vi "2636 Pulse Generator.vi"() -> ()   [LabVIEW 2023]
uses:
  <instrlib>/Keithley 2600 Series/Public/Channel.ctl
  <instrlib>/Keithley 2600 Series/Keithley 2600 Series.lvlib
  <userlib>/_OpenG.lib/time/time.llb/openg_time.lvlib
panel:
  in  "Pulse Number":u32=10
  out "Gate Pulse":cluster{"X":dbl[], "Y":dbl[]}[](graph)
  in  "error in (no error)":errorcluster
  in  "Auto Enable Output":bool=TRUE
  in  "Reset":bool=TRUE
  in  "Error Query":bool
  out "error out":errorcluster
  out "Complete?":bool
  in  "Stop":bool
  in  "Pulse Duration (s)":dbl=0.01
  in  "Post-Pulse Duration (s)":dbl=0.05
  in  "Pre-Pulse Duration (s)":dbl=0.05
  in  "Pulse Level (V)":dbl=15.0
  in  "Pulse Channel":T1
  in  "2636 Address":refnum<visa-resource-name>="GPIB0::26::INSTR"
  # "Pulse Generator"
  # "by JHC (20250611)"
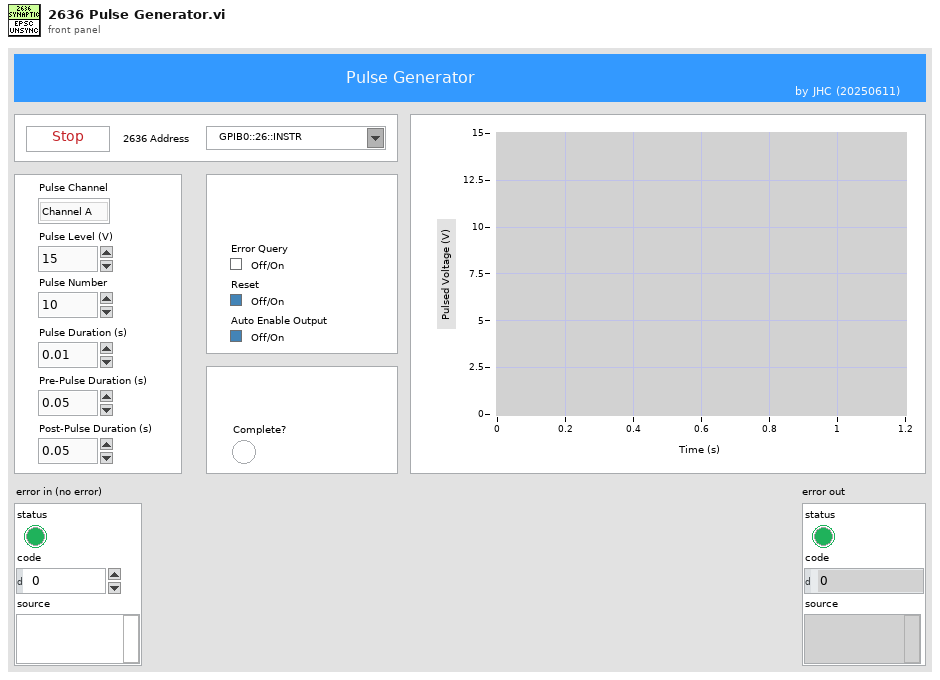
[diagram p1: front panel]
types:
  T1 = typedef "Keithley 2600 Series.lvlib/Channel.ctl" = enum32{"Channel A", "Channel B"}
  T2 = enum16{"None/Disconnect", "Digital I/O Trigger", "TSP-Link Trigger", "LAN Trigger", "Blender", "Timer Expired", "Front Panel Trigger", "Software Trigger", "SMU Sweeping", "SMU Armed", "SMU Source Complete", "SMU Measure Complete", "SMU Pulse Complete", "SMU Sweep Complete", "SMU Idle"}
  T3 = enum16{"Current", "Voltage", "IV", "Resistance", "Power"}
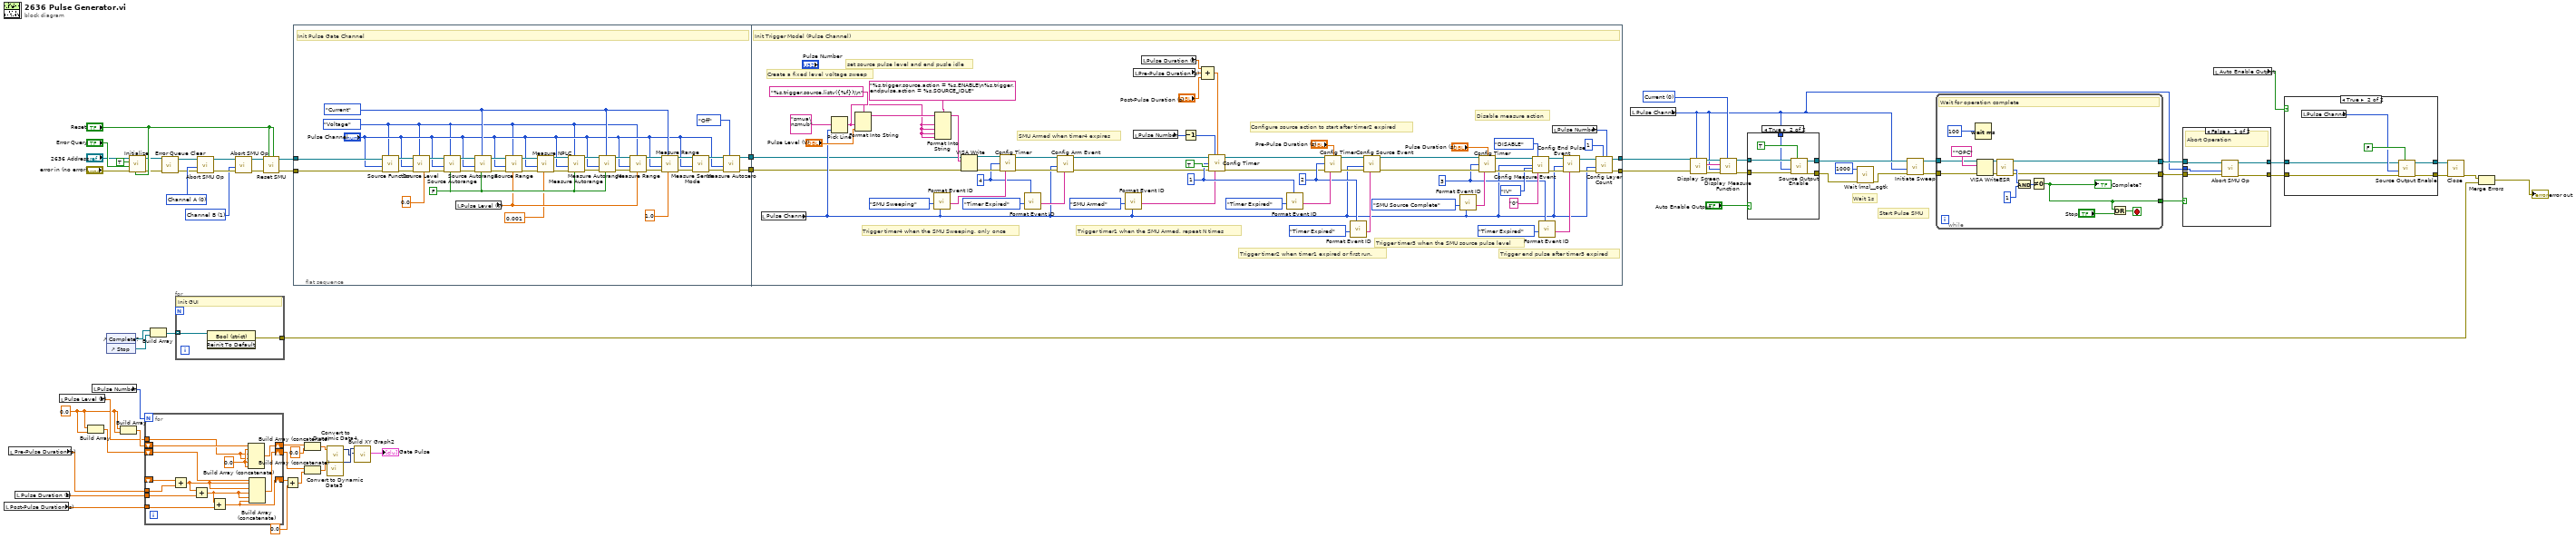
[diagram p0: block diagram]
diagram:
  w6 = 0.0 ("element")
  w42 = u16 1 items=["Channel A", "Channel B"] ("Channel (Channel A)")
  w43 = u16 0 items=["Channel A", "Channel B"] ("Channel (Channel A)")
  w52 = u16 0 items=["Current", "Voltage", "Resistance", "Power"] ("Function (Current)")
  # "Wait 1s"
  # "Start Pulse SMU"
  n1 = local read "Post-Pulse Duration (s)"() -> (w19:dbl)
  n2 = local read "Pre-Pulse Duration (s)"() -> (w22:dbl)
  n3 = local read "Pulse Duration (s)"() -> (w20:dbl)
  n4 = local read "Pulse Level (V)"() -> (w21:dbl)
  n5 = Build Array(w6, w6) -> (w24:dbl[])
  n6 = local read "Pulse Number"() -> (w25:u32)
  n7 = control-ref of="Complete?"() -> (w50:refnum<vi>)
  n8 = control-ref of="Stop"() -> (w48:refnum<vi>)
  n9 = Build Array(w6, w6) -> (w23:dbl[])
  n10 = call <instrlib>:"Initialize.vi"("Reset (True)"="Reset", "error in (no error)"="error in (no error)", "Error Query (False)"="Error Query", "ID Query (True)"=TRUE, "VISA resource name"="2636 Address") -> ("error out"=w27:errorcluster, "VISA resource name out"=w30:refnum<visa-resource-name>)  [unwired: 5 in]
  n11 = for {
    N: w25 -> [_]
    shift-right: [w77] -> w18
    shift-left: w23 -> [w78]
    shift-right: [w79] -> w17
    shift-left: w24 -> [w80]
    tunnel: w22 -> [w74]
    tunnel: w21 -> [w69]
    tunnel: w20 -> [w76]
    shift-right: [w71] -> w10
    shift-left: _ -> [w81]
    tunnel: w19 -> [w75]
    w73 = 0.0 ("element")
    n12 = Add(x=w81, y=w74) -> (x+y=w72:dbl)
    n13 = Add(x=w72, y=w76) -> (x+y=w70:dbl)
    n14 = Add(x=w70, y=w75) -> (x+y=w71:dbl)
    n15 = Build Array (concatenate)(w78, w73, w69, w69, w73, w73) -> (w77:dbl[])
    n16 = Build Array (concatenate)(w80, w72, w72, w70, w70, w71) -> (w79:dbl[])
  }
  n17 = Build Array(w50, w48) -> (w49:refnum<vi>[])
  n18 = call <instrlib>:"Error Queue Clear.vi"("error in (no error)"=w27, "VISA resource name"=w30) -> ("error out"=w28:errorcluster, "VISA resource name out"=w29:refnum<visa-resource-name>)  [unwired: 6 in, 2 out]
  n19 = for {
    tunnel: w49 -> [w83] mode=indexing
    tunnel: [w82] -> w5
    # "Init GUI"
    n20 = invoke class="Bool (strict)" method="Reinit To Default"(reference=w83) -> (error out=w82:errorcluster)  [unwired: 2 in, 2 out]
  }
  n21 = call <instrlib>:"Abort SMU Op.vi"("error in"=w28, "Channel (Channel A)"=w43, "VISA resource name"=w29) -> ("error out"=w44:errorcluster, "VISA resource name out"=w45:refnum<visa-resource-name>)  [unwired: 5 in, 2 out]
  n22 = call <instrlib>:"Abort SMU Op.vi"("error in"=w44, "Channel (Channel A)"=w42, "VISA resource name"=w45) -> ("error out"=w40:errorcluster, "VISA resource name out"=w41:refnum<visa-resource-name>)  [unwired: 5 in, 2 out]
  n23 = call <instrlib>:"Reset SMU.vi"("SMU B (No)"="Reset", "SMU A (No)"="Reset", "error in (no error)"=w40, "VISA resource name"=w41) -> ("error out"=w67:errorcluster, "VISA resource name out"=w68:refnum<visa-resource-name>)  [unwired: 4 in, 2 out]
  n24 = Add(x=w10, y=0.0) -> (x+y=w9:dbl)
  n25 = flat-sequence {
    tunnel: w68 -> [w116]
    tunnel: w67 -> [w115]
    tunnel: [w85] -> w8
    tunnel: [w84] -> w7
    tunnel: w8 -> [w122]
    tunnel: w7 -> [w121]
    tunnel: [w120] -> w3
    tunnel: [w119] -> w2
    frame #0 {
      w105 = enum32{"Current", "Voltage"}."Current" ("Function (Current)")
      w106 = FALSE ("Autorange (On)")
      w89 = enum32{"Current", "Voltage"}."Voltage" ("Function (Current)")
      # "Init Pulse Gate Channel"
      n26 = call <instrlib>:"Source Function.vi"("Function (Current)"=w89, "error in (no error)"=w115, "Channel (Channel A)"="Pulse Channel", "VISA resource name"=w116) -> ("error out"=w117:errorcluster, "VISA resource name out"=w118:refnum<visa-resource-name>)  [unwired: 4 in, 2 out]
      n27 = call <instrlib>:"Source Level.vi"("Level (0.000)"=0.0, "Function (Current)"=w89, "error in (no error)"=w117, "Channel (Channel A)"="Pulse Channel", "VISA resource name"=w118) -> ("error out"=w113:errorcluster, "VISA resource name out"=w114:refnum<visa-resource-name>)  [unwired: 3 in, 2 out]
      n28 = call <instrlib>:"Source Autorange.vi"("Autorange (On)"=w106, "Function (Current)"=w89, "error in (no error)"=w113, "Channel (Channel A)"="Pulse Channel", "VISA resource name"=w114) -> ("error out"=w111:errorcluster, "VISA resource name out"=w112:refnum<visa-resource-name>)  [unwired: 3 in, 2 out]
      n29 = local read "Pulse Level (V)"() -> (w88:dbl)
      n30 = call <instrlib>:"Source Autorange.vi"("Autorange (On)"=w106, "Function (Current)"=w105, "error in (no error)"=w111, "Channel (Channel A)"="Pulse Channel", "VISA resource name"=w112) -> ("error out"=w96:errorcluster, "VISA resource name out"=w98:refnum<visa-resource-name>)  [unwired: 3 in, 2 out]
      n31 = call <instrlib>:"Source Range.vi"("Range (1.000)"=w88, "Function (Current)"=w89, "error in (no error)"=w96, "Channel (Channel A)"="Pulse Channel", "VISA resource name"=w98) -> ("error out"=w95:errorcluster, "VISA resource name out"=w97:refnum<visa-resource-name>)  [unwired: 3 in, 2 out]
      n32 = call <instrlib>:"Measure NPLC.vi"("NPLC (1.000)"=0.001, "error in (no error)"=w95, "Channel (Channel A)"="Pulse Channel", "VISA resource name"=w97) -> ("error out"=w110:errorcluster, "VISA resource name out"=w107:refnum<visa-resource-name>)  [unwired: 4 in, 2 out]
      n33 = call <instrlib>:"Measure Autorange.vi"("Autorange (On)"=w106, "Function (Current)"=w89, "error in (no error)"=w110, "Channel (Channel A)"="Pulse Channel", "VISA resource name"=w107) -> ("error out"=w109:errorcluster, "VISA resource name out"=w108:refnum<visa-resource-name>)  [unwired: 3 in, 2 out]
      n34 = call <instrlib>:"Measure Autorange.vi"("Autorange (On)"=w106, "Function (Current)"=w105, "error in (no error)"=w109, "Channel (Channel A)"="Pulse Channel", "VISA resource name"=w108) -> ("error out"=w94:errorcluster, "VISA resource name out"=w93:refnum<visa-resource-name>)  [unwired: 3 in, 2 out]
      n35 = call <instrlib>:"Measure Range.vi"("Range (1.000)"=w88, "Function (Current)"=w89, "error in (no error)"=w94, "Channel (Channel A)"="Pulse Channel", "VISA resource name"=w93) -> ("error out"=w91:errorcluster, "VISA resource name out"=w92:refnum<visa-resource-name>)  [unwired: 3 in, 2 out]
      n36 = call <instrlib>:"Measure Range.vi"("Range (1.000)"=1.0, "Function (Current)"=w105, "error in (no error)"=w91, "Channel (Channel A)"="Pulse Channel", "VISA resource name"=w92) -> ("error out"=w104:errorcluster, "VISA resource name out"=w103:refnum<visa-resource-name>)  [unwired: 3 in, 2 out]
      n37 = call <instrlib>:"Measure Sense Mode.vi"("error in (no error)"=w104, "Channel (Channel A)"="Pulse Channel", "VISA resource name"=w103) -> ("error out"=w101:errorcluster, "VISA resource name out"=w102:refnum<visa-resource-name>)  [unwired: 2 in, 5 out]
      n38 = call <instrlib>:"Measure Autozero.vi"("Autozero (Auto)"=enum32{"Off", "Once", "Auto"}."Off", "error in (no error)"=w101, "Channel (Channel A)"="Pulse Channel", "VISA resource name"=w102) -> ("error out"=w84:errorcluster, "VISA resource name out"=w85:refnum<visa-resource-name>)  [unwired: 1 in, 5 out]
    }
    frame #1 {
      w130 = u32 4 ("Timer Number (1)")
      w141 = u32 1 ("Timer Number (1)")
      w153 = u32 3 ("Timer Number (1)")
      w173 = u32 2 ("Timer Number (1)")
      # "SMU Armed when timer4 expires"
      # "Trigger timer4 when the SMU Sweeping, only once"
      # "Trigger timer1 when the SMU Armed, repeat N times"
      # "Trigger end pulse after timer3 expired"
      # "Disable measure action"
      # "set source pulse level and end pusle idle"
      # "Trigger timer3 when the SMU source pulse level"
      # "Create a fixed level voltage sweep"
      # "Configure source action to start after timer2 expired"
      # "Trigger timer2 when timer1 expired or first run."
      # "Init Trigger Model (Pulse Channel)"
      n39 = local read "Pulse Channel"() -> (w126:T1)
      n40 = Pick Line(multi-line string="smua\nsmub", line index=w126) -> (output string=w138:string)  [unwired: 1 in]
      n41 = Format Into String(format string="%s.trigger.source.listv({%f})\\n", w138, "Pulse Level (V)") -> (resulting string=w170:string)  [unwired: 2 in, 1 out]
      n42 = call <instrlib>:"Format Event ID.vi"("Channel (Channel A)"=w126, "Event Type (None)"=T2."SMU Sweeping") -> ("Event ID"=w133:string)  [unwired: 8 in, 1 out]
      n43 = Format Into String(format string="%s.trigger.source.action = %s.ENABLE\n%s.trigger.endpulse.action = %s.SOURCE_IDLE", initial string=w170, w138, w138, w138, w138) -> (resulting string=w167:string)  [unwired: 1 in, 1 out]
      n44 = VISA Write(VISA resource name=w122, write buffer=w167, error in (no error)=w121) -> (VISA resource name out=w135:refnum<visa-resource-name>, error out=w134:errorcluster)  [unwired: 1 out]
      n45 = call <instrlib>:"Config Timer.vi"("VISA resource name"=w135, "Timer Number (1)"=w130, "error in"=w134, "Input Event"=w133) -> ("VISA resource name out"=w132:refnum<visa-resource-name>, "error out"=w128:errorcluster)  [unwired: 8 in, 2 out]
      n46 = call <instrlib>:"Format Event ID.vi"("Event Module # (1)"=w130, "Event Type (None)"=T2."Timer Expired") -> ("Event ID"=w129:string)  [unwired: 8 in, 1 out]
      n47 = call <instrlib>:"Config Arm Event.vi"("Arm Input Event"=w129, "error in"=w128, "Channel (Channel A)"=w126, "VISA resource name"=w132) -> ("error out"=w124:errorcluster, "VISA resource name out"=w123:refnum<visa-resource-name>)  [unwired: 4 in, 2 out]
      n48 = call <instrlib>:"Format Event ID.vi"("Channel (Channel A)"=w126, "Event Type (None)"=T2."SMU Armed") -> ("Event ID"=w125:string)  [unwired: 8 in, 1 out]
      n49 = local read "Pre-Pulse Duration (s)"() -> (w150:dbl)
      n50 = local read "Pulse Number"() -> (w146:u32)
      n51 = local read "Pulse Duration (s)"() -> (w151:dbl)
      n52 = Decrement(x=w146) -> (x-1=w142:u32)
      n53 = Compound Arithmetic op=ADD(w151, w150, "Post-Pulse Duration (s)") -> (w148:dbl)
      n54 = call <instrlib>:"Config Timer.vi"("VISA resource name"=w123, "Count (1)"=w142, "Delay (1e-3)"=w148, "Timer Number (1)"=w141, "Passthrough (Off)"=TRUE, "error in"=w124, "Input Event"=w125) -> ("VISA resource name out"=w143:refnum<visa-resource-name>, "error out"=w144:errorcluster)  [unwired: 5 in, 2 out]
      n55 = call <instrlib>:"Format Event ID.vi"("Event Module # (1)"=w141, "Event Type (None)"=T2."Timer Expired") -> ("Event ID"=w177:string)  [unwired: 8 in, 1 out]
      n56 = call <instrlib>:"Config Timer.vi"("VISA resource name"=w143, "Delay (1e-3)"="Pre-Pulse Duration (s)", "Timer Number (1)"=w173, "error in"=w144, "Input Event"=w177) -> ("VISA resource name out"=w176:refnum<visa-resource-name>, "error out"=w175:errorcluster)  [unwired: 7 in, 2 out]
      n57 = call <instrlib>:"Format Event ID.vi"("Event Module # (1)"=w173, "Event Type (None)"=T2."Timer Expired") -> ("Event ID"=w172:string)  [unwired: 8 in, 1 out]
      n58 = call <instrlib>:"Config Source Event.vi"("Input Event"=w172, "error in"=w175, "Channel (Channel A)"=w126, "VISA resource name"=w176) -> ("error out"=w162:errorcluster, "VISA resource name out"=w163:refnum<visa-resource-name>)  [unwired: 4 in, 2 out]
      n59 = call <instrlib>:"Format Event ID.vi"("Channel (Channel A)"=w126, "Event Type (None)"=T2."SMU Source Complete") -> ("Event ID"=w165:string)  [unwired: 8 in, 1 out]
      n60 = call <instrlib>:"Config Timer.vi"("VISA resource name"=w163, "Delay (1e-3)"="Pulse Duration (s)", "Timer Number (1)"=w153, "error in"=w162, "Input Event"=w165) -> ("VISA resource name out"=w161:refnum<visa-resource-name>, "error out"=w160:errorcluster)  [unwired: 7 in, 2 out]
      n61 = call <instrlib>:"Config Measure Event.vi"("VISA resource name"=w161, "Configure Measurement (Disable)"=enum8{"DISABLE", "ENABLE", "ASYNC"}."DISABLE", "Channel (Channel A)"=w126, "Function (Current)"=T3."IV", "error in"=w160, "Measure Input Event"="0") -> ("VISA resource name out"=w156:refnum<visa-resource-name>, "error out"=w155:errorcluster)  [unwired: 6 in, 2 out]
      n62 = call <instrlib>:"Format Event ID.vi"("Event Module # (1)"=w153, "Event Type (None)"=T2."Timer Expired") -> ("Event ID"=w152:string)  [unwired: 8 in, 1 out]
      n63 = local read "Pulse Number"() -> (w136:u32)
      n64 = call <instrlib>:"Config End Pulse Event.vi"("Input Event"=w152, "error in"=w155, "Channel (Channel A)"=w126, "VISA resource name"=w156) -> ("error out"=w140:errorcluster, "VISA resource name out"=w139:refnum<visa-resource-name>)  [unwired: 4 in, 2 out]
      n65 = call <instrlib>:"Config Layer Count.vi"("Trigger Count (1)"=w136, "Arm Count (1)"=u32 1 ("Trigger Count (1)"), "error in"=w140, "Channel (Channel A)"=w126, "VISA resource name"=w139) -> ("error out"=w119:errorcluster, "VISA resource name out"=w120:refnum<visa-resource-name>)  [unwired: 3 in, 2 out]
    }
  }
  n66 = Build Array (concatenate)(w18, 0.0 ("element")) -> (w15:dbl[])
  n67 = Build Array (concatenate)(w17, w9) -> (w14:dbl[])
  n68 = call "Convert to Dynamic Data5"("Array"=w14) -> ("Dynamic Data Type"=w12:dynamicdata)  [unwired: 3 in]
  n69 = call "Convert to Dynamic Data4"("Array"=w15) -> ("Dynamic Data Type"=w11:dynamicdata)  [unwired: 3 in]
  n70 = call "Build XY Graph2"("Y Input"=w11, "X Input"=w12) -> ("XY Graph"=→"Gate Pulse":cluster{"X":dbl[], "Y":dbl[]}[])  [unwired: 8 in, 1 out]
  n71 = local read "Pulse Channel"() -> (w1:T1)
  n72 = call <instrlib>:"Display Screen.vi"("Screen (Channels A & B)"=w1, "error in (no error)"=w2, "VISA resource name"=w3) -> ("error out"=w57:errorcluster, "Node Out"=w56:string, "VISA resource name out"=w55:refnum<visa-resource-name>)  [unwired: 5 in, 1 out]
  n73 = call <instrlib>:"Display Measure Function.vi"("Function (Current)"=w52, "error in (no error)"=w57, "Channel (Channel A)"=w1, "Node In"=w56, "VISA resource name"=w55) -> ("error out"=w54:errorcluster, "VISA resource name out"=w53:refnum<visa-resource-name>)  [unwired: 3 in, 2 out]
  n74 = case shown="True" "Auto Enable Output" {
    tunnel: [w181 w188] -> w34
    tunnel: [w182 w187] -> w35
    tunnel: w54 -> [w181 w186]
    tunnel: w1 -> [_ w183]
    tunnel: w53 -> [w182 w185]
    frame False {
    }
    frame True {
      n75 = call <instrlib>:"Source Output Enable.vi"("Output (Off)"=TRUE, "error in (no error)"=w186, "Channel (Channel A)"=w183, "VISA resource name"=w185) -> ("error out"=w188:errorcluster, "VISA resource name out"=w187:refnum<visa-resource-name>)  [unwired: 4 in, 2 out]
    }
  }
  n76 = call <userlib>:"Wait (ms)__ogtk.vi"("error in (no error)"=w34, "milliseconds to wait"=u32 1000) -> ("error out"=w33:errorcluster)  [unwired: 8 in, 1 out]
  n77 = call <instrlib>:"Initiate Sweep.vi"("error in"=w33, "Channel (Channel A)"=w1, "VISA resource name"=w35) -> ("error out"=w66:errorcluster, "VISA resource name out"=w65:refnum<visa-resource-name>)  [unwired: 5 in, 2 out]
  n78 = while {
    tunnel: w65 -> [w192]
    tunnel: w66 -> [w191]
    tunnel: [w190] -> w64
    tunnel: [w189] -> w63
    tunnel: [w193] -> w58
    stop <- w194 stop-if-true
    # "Wait for operation complete"
    n79 = Wait (ms)(milliseconds to wait=u32 100) -> ()  [unwired: 1 out]
    n80 = VISA Write(VISA resource name=w192, write buffer="*OPC", error in (no error)=w191) -> (VISA resource name out=w201:refnum<visa-resource-name>, error out=w200:errorcluster)  [unwired: 1 out]
    n81 = call <instrlib>:"ESR.vi"("error in (no error)"=w200, "VISA resource name"=w201) -> ("error out"=w189:errorcluster, "ESR"=w199:u8, "VISA resource name out"=w190:refnum<visa-resource-name>)  [unwired: 5 in, 2 out]
    n82 = And(x=w199, y=u8 1) -> (x .and. y?=w198:u8)
    n83 = Not Equal To 0?(x=w198) -> (x != 0?=w193:bool)
    "Complete?" <- w193
    n84 = Or(x=w193, y="Stop") -> (x .or. y?=w194:bool)
  }
  n85 = case shown="False" w58 {
    tunnel: w64 -> [w207 w209]
    tunnel: w63 -> [w206 w208]
    tunnel: [w205 w209] -> w62
    tunnel: [w204 w208] -> w61
    tunnel: w1 -> [w203 _]
    frame False {
      # "Abort Operation"
      n86 = call <instrlib>:"Abort SMU Op.vi"("error in"=w206, "Channel (Channel A)"=w203, "VISA resource name"=w207) -> ("error out"=w204:errorcluster, "VISA resource name out"=w205:refnum<visa-resource-name>)  [unwired: 5 in, 2 out]
    }
    frame True {
      # "Operation Completed"
    }
  }
  n87 = local read "Auto Enable Output"() -> (w36:bool)
  n88 = case shown="True" w36 {
    tunnel: w62 -> [w211 w215]
    tunnel: w61 -> [w210 w214]
    tunnel: [w210 w213] -> w60
    tunnel: [w211 w212] -> w59
    frame False {
    }
    frame True {
      n89 = local read "Pulse Channel"() -> (w216:T1)
      n90 = call <instrlib>:"Source Output Enable.vi"("Output (Off)"=FALSE, "error in (no error)"=w214, "Channel (Channel A)"=w216, "VISA resource name"=w215) -> ("error out"=w213:errorcluster, "VISA resource name out"=w212:refnum<visa-resource-name>)  [unwired: 4 in, 2 out]
    }
  }
  n91 = call <instrlib>:"Close.vi"("error in (no error)"=w60, "VISA resource name"=w59) -> ("error out"=w47:errorcluster)  [unwired: 9 in]
  n92 = Merge Errors(w47, w5) -> (→"error out":errorcluster)
